vi "UMLEditor menuUpdates.vi"(0 "menu":refnum<k9>, 1 "menuAction":T1, 2 "item":string, 3 "addfirst(false)":bool, 5 "error in (no error)":errorcluster) -> (19 "error out":errorcluster)   [LabVIEW 2020]
doc: "Gets current diagram values"
uses:
  <resource>/Framework/Providers/Open_GDS/UML/UMLEditor/UMLEditor MenuActionType.ctl
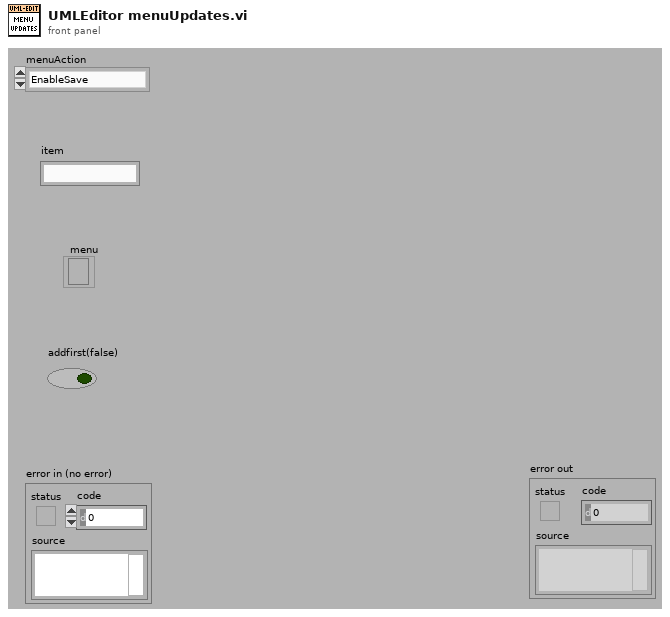
[diagram p1: front panel]
types:
  T1 = typedef "UMLEditor MenuActionType.ctl" = enum16{"EnableSave", "EnablePaste", "DisablePaste", "DiableSave", "AddRecentFile", "disablePropDel", "enablePropDel", "enablePropDisDel", "diasbleClassRel", "enableClassRel", "Class", "State", "Other", "EnableXMI", "DisableXMI", "EnableCopy", "DisableCopy"}
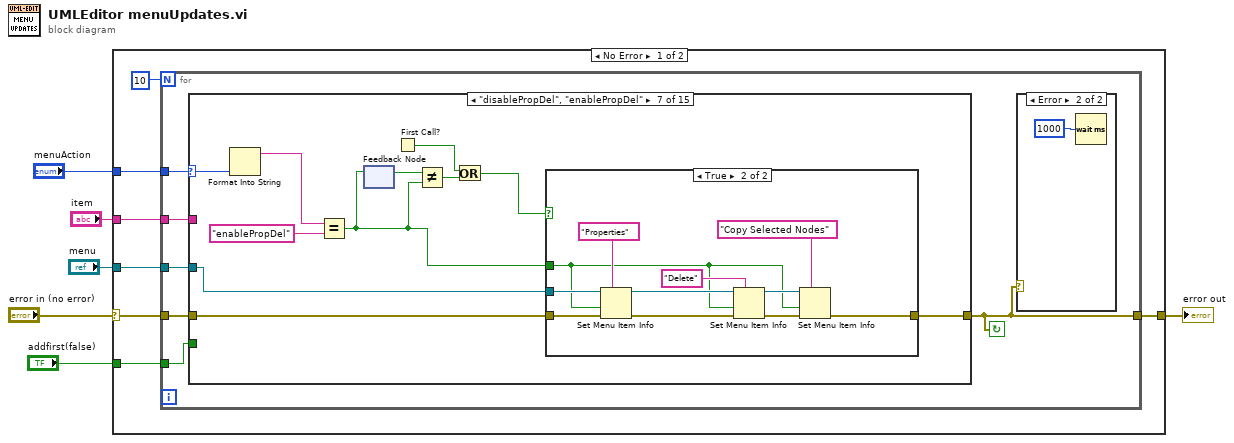
[diagram p0: block diagram]
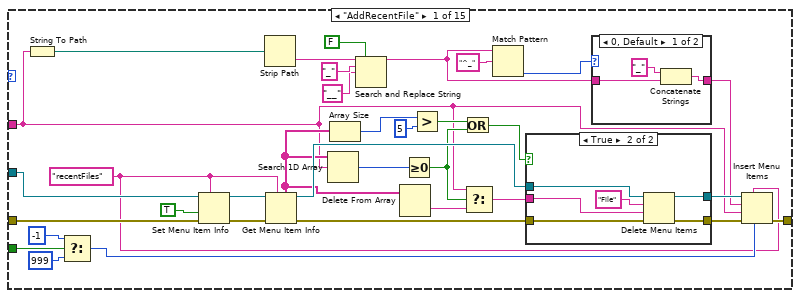
[diagram p3: hidden frame]
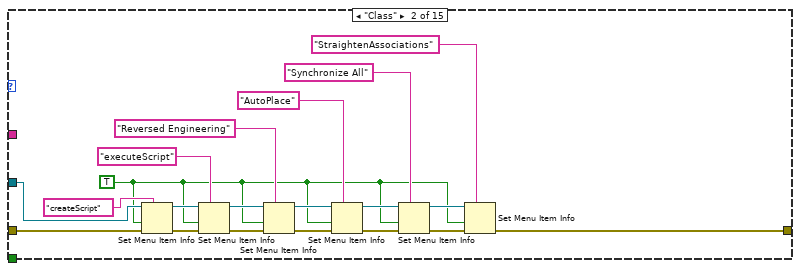
[diagram p6: hidden frame]
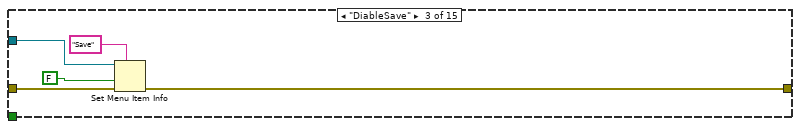
[diagram p7: hidden frame]
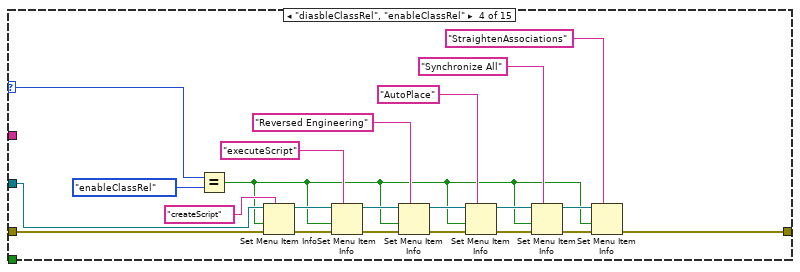
[diagram p8: hidden frame]
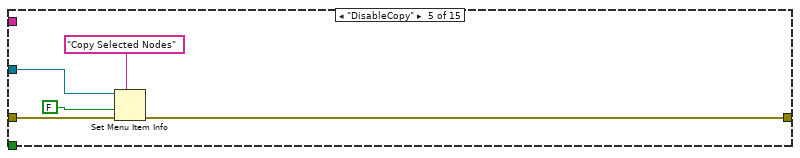
[diagram p9: hidden frame]
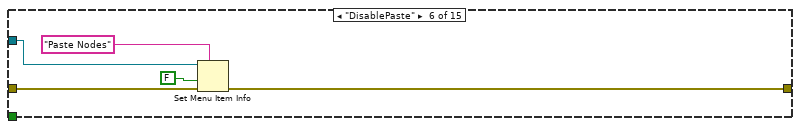
[diagram p10: hidden frame]
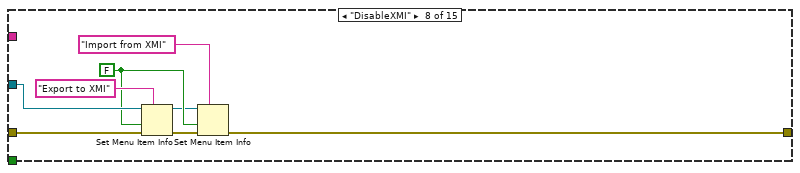
[diagram p12: hidden frame]
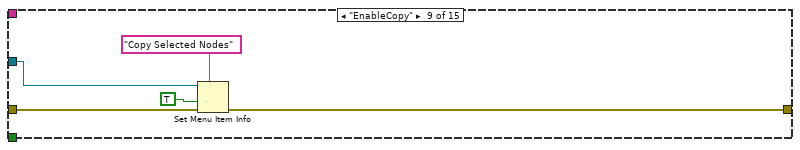
[diagram p13: hidden frame]
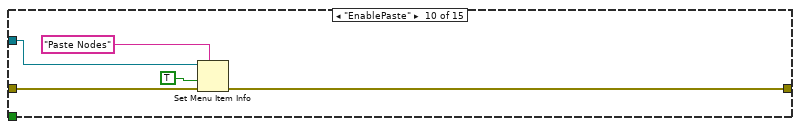
[diagram p14: hidden frame]
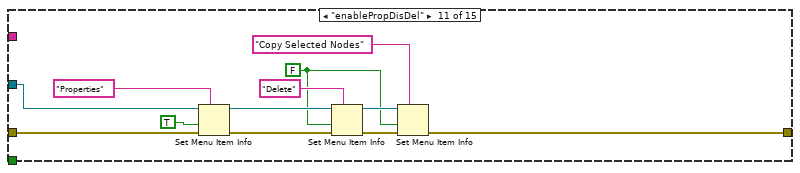
[diagram p15: hidden frame]
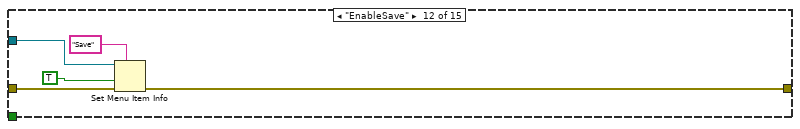
[diagram p16: hidden frame]
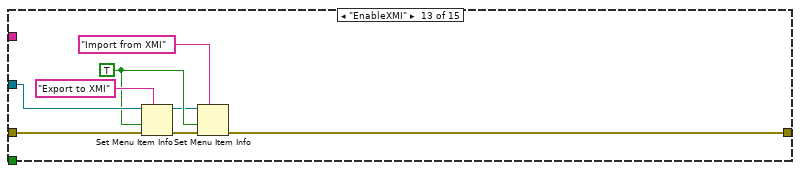
[diagram p17: hidden frame]
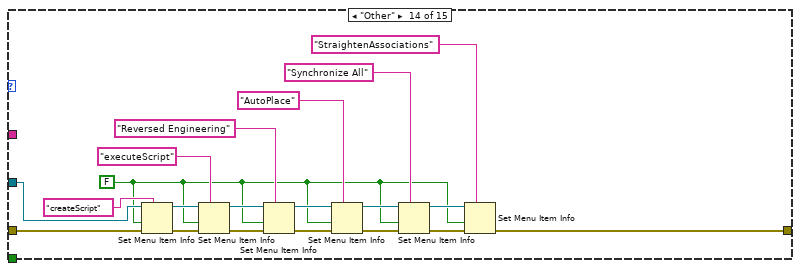
[diagram p18: hidden frame]
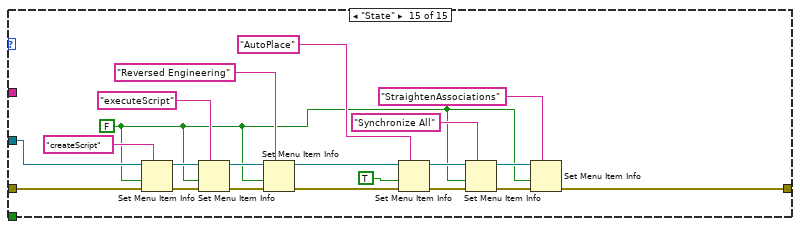
[diagram p19: hidden frame]
diagram:
  n1 = case shown="No Error" "error in (no error)" {
    selector: "error in (no error)" -> [w13 w231]
    tunnel: [w12 w231] -> w5
    tunnel: "menuAction" -> [w11 _]
    tunnel: "item" -> [w10 _]
    tunnel: "addfirst(false)" -> [w9 _]
    tunnel: "menu" -> [w8 _]
    frame No Error {
      n2 = for {
        N: 10 -> [_]
        tunnel: w11 -> [w18]
        tunnel: w10 -> [w17]
        tunnel: w9 -> [w16]
        tunnel: w8 -> [w15]
        tunnel: w13 -> [w19]
        tunnel: [w14] -> w12
        stop <- w14 continue-if-true
        n3 = case shown="\"disablePropDel\", \"enablePropDel\"" w18 {
          selector: w18 -> [_ _ _ w94 _ _ w125 _ _ _ _ _ _ _ _]
          tunnel: w15 -> [w34 w86 w91 w113 w118 w123 w134 w154 w159 w164 w176 w181 w189 w209 w230]
          tunnel: w19 -> [w32 w85 w90 w112 w117 w122 w133 w153 w158 w163 w175 w180 w188 w208 w229]
          tunnel: [w54 w68 w89 w95 w116 w121 w132 w150 w157 w162 w166 w179 w184 w191 w212] -> w14
          tunnel: w17 -> [w41 _ _ _ _ _ _ _ _ _ _ _ _ _ _]
          tunnel: w16 -> [w38 _ _ _ _ _ _ _ _ _ _ _ _ _ _]
          frame "AddRecentFile" {
            w30 = "recentFiles" ("menu tag")
            n4 = String To Path(string=w41) -> (path=w53:path)
            n5 = Select(t=-1, s=w38, f=999) -> (s? t:f=w36:i32)
            n6 = Set Menu Item Info(7:w30, 8:w32, 9:TRUE ("enabled"), 11:w34) -> (0:w31:errorcluster, 3:w33:refnum<k9>)  [unwired: 3 out]
            n7 = Strip Path(path=w53) -> (name=w28:string)  [unwired: 1 out]
            n8 = Get Menu Item Info(7:w30, 8:w31, 11:w33) -> (0:w48:errorcluster, 3:w50:refnum<k9>, 5:w46:string[])  [unwired: 4 out]
            n9 = Search 1D Array(1D array=w46, element=w41) -> (index of element=w43:i32)  [unwired: 1 out]
            n10 = Array Size(array=w46) -> (size(s)=w52:i32)
            n11 = Search and Replace String(replace all?=FALSE ("replace all? (F)"), input string=w28, search string="_", replace string="__" ("replace string (\"\")")) -> (result string=w22:string)  [unwired: 1 in, 6 out]
            n12 = Delete From Array(array=w46) -> (deleted portion=w40:string)  [unwired: 2 in, 1 out]
            n13 = Greater Or Equal To 0?(x=w43) -> (x >= 0?=w42:bool)
            n14 = Greater?(x=w52, y=5) -> (0:w44:bool)
            n15 = Or(x=w44, y=w42) -> (x .or. y?=w45:bool)
            n16 = Select(t=w41, s=w42, f=w40) -> (s? t:f=w39:string)
            n17 = Match Pattern(string=w22, regular expression="^_") -> (offset past match=w23:i32)  [unwired: 4 out]
            n18 = case shown="True" w45 {
              tunnel: w50 -> [w60 w66]
              tunnel: [w60 w65] -> w49
              tunnel: w39 -> [_ w62]
              tunnel: w48 -> [w59 w64]
              tunnel: [w59 w63] -> w47
              frame False {
              }
              frame True {
                n19 = Delete Menu Items(6:w64, 7:w62, 8:"File" ("menu tag"), 9:w66) -> (0:w63:errorcluster, 3:w65:refnum<k9>)
              }
            }
            n20 = case shown="0, Default" w23 {
              tunnel: w22 -> [w57 w58]
              tunnel: [w56 w58] -> w21
              frame 0, Default {
                n21 = Concatenate Strings("_" ("search string"), w57) -> (w56:string)
              }
              frame -1 {
              }
            }
            n22 = Insert Menu Items(4:w36, 5:w30, 6:w47, 7:w41, 8:w21, 9:w49) -> (0:w54:errorcluster)  [unwired: 2 out]
          }
          frame "Class" {
            w67 = TRUE ("enabled")
            n23 = Set Menu Item Info(7:"createScript" ("item tag"), 8:w85, 9:w67, 11:w86) -> (0:w81:errorcluster, 3:w83:refnum<k9>)  [unwired: 3 out]
            n24 = Set Menu Item Info(7:"executeScript" ("item tag"), 8:w81, 9:w67, 11:w83) -> (0:w77:errorcluster, 3:w80:refnum<k9>)  [unwired: 3 out]
            n25 = Set Menu Item Info(7:"Reversed Engineering" ("item tag"), 8:w77, 9:w67, 11:w80) -> (0:w79:errorcluster, 3:w78:refnum<k9>)  [unwired: 3 out]
            n26 = Set Menu Item Info(7:"AutoPlace" ("item tag"), 8:w79, 9:w67, 11:w78) -> (0:w73:errorcluster, 3:w72:refnum<k9>)  [unwired: 3 out]
            n27 = Set Menu Item Info(7:"Synchronize All" ("item tag"), 8:w73, 9:w67, 11:w72) -> (0:w69:errorcluster, 3:w70:refnum<k9>)  [unwired: 3 out]
            n28 = Set Menu Item Info(7:"StraightenAssociations" ("item tag"), 8:w69, 9:w67, 11:w70) -> (0:w68:errorcluster)  [unwired: 4 out]
          }
          frame "DiableSave" {
            n29 = Set Menu Item Info(7:"Save" ("item tag"), 8:w90, 9:FALSE ("enabled"), 11:w91) -> (0:w89:errorcluster)  [unwired: 4 out]
          }
          frame "diasbleClassRel", "enableClassRel" {
            n30 = Equal?(x=w94, y=UMLEditor_MenuActionType."enableClassRel") -> (x = y?=w92:bool)
            n31 = Set Menu Item Info(7:"createScript" ("item tag"), 8:w112, 9:w92, 11:w113) -> (0:w108:errorcluster, 3:w110:refnum<k9>)  [unwired: 3 out]
            n32 = Set Menu Item Info(7:"executeScript" ("item tag"), 8:w108, 9:w92, 11:w110) -> (0:w104:errorcluster, 3:w107:refnum<k9>)  [unwired: 3 out]
            n33 = Set Menu Item Info(7:"Reversed Engineering" ("item tag"), 8:w104, 9:w92, 11:w107) -> (0:w106:errorcluster, 3:w105:refnum<k9>)  [unwired: 3 out]
            n34 = Set Menu Item Info(7:"AutoPlace" ("item tag"), 8:w106, 9:w92, 11:w105) -> (0:w100:errorcluster, 3:w99:refnum<k9>)  [unwired: 3 out]
            n35 = Set Menu Item Info(7:"Synchronize All" ("item tag"), 8:w100, 9:w92, 11:w99) -> (0:w96:errorcluster, 3:w97:refnum<k9>)  [unwired: 3 out]
            n36 = Set Menu Item Info(7:"StraightenAssociations" ("item tag"), 8:w96, 9:w92, 11:w97) -> (0:w95:errorcluster)  [unwired: 4 out]
          }
          frame "DisableCopy" {
            n37 = Set Menu Item Info(7:"Copy Selected Nodes" ("item tag"), 8:w117, 9:FALSE ("enabled"), 11:w118) -> (0:w116:errorcluster)  [unwired: 4 out]
          }
          frame "DisablePaste" {
            n38 = Set Menu Item Info(7:"Paste Nodes" ("item tag"), 8:w122, 9:FALSE ("enabled"), 11:w123) -> (0:w121:errorcluster)  [unwired: 4 out]
          }
          frame "disablePropDel", "enablePropDel" {
            n39 = Format Into String(w125) -> (resulting string=w124:string)  [unwired: 3 in, 1 out]
            n40 = Equal?(x=w124, y="enablePropDel") -> (x = y?=w129:bool)
            n41 = feedback-in #1(w129) -> ()
            n42 = feedback #1() -> (w130:bool)  [unwired: 1 in]
            n43 = First Call?() -> (First Call?: T/F=w127:bool)
            n44 = Not Equal?(x=w130, y=w129) -> (x != y?=w128:bool)
            n45 = Or(x=w127, y=w128) -> (x .or. y?=w126:bool)
            n46 = case shown="True" w126 {
              tunnel: w134 -> [_ w146]
              tunnel: w133 -> [w135 w145]
              tunnel: [w135 w138] -> w132
              tunnel: w129 -> [_ w136]
              frame False {
              }
              frame True {
                n47 = Set Menu Item Info(7:"Properties" ("item tag"), 8:w145, 9:w136, 11:w146) -> (0:w141:errorcluster, 3:w143:refnum<k9>)  [unwired: 3 out]
                n48 = Set Menu Item Info(7:"Delete" ("item tag"), 8:w141, 9:w136, 11:w143) -> (0:w140:errorcluster, 3:w139:refnum<k9>)  [unwired: 3 out]
                n49 = Set Menu Item Info(7:"Copy Selected Nodes" ("item tag"), 8:w140, 9:w136, 11:w139) -> (0:w138:errorcluster)  [unwired: 4 out]
              }
            }
          }
          frame "DisableXMI" {
            w148 = FALSE ("enabled")
            n50 = Set Menu Item Info(7:"Export to XMI" ("item tag"), 8:w153, 9:w148, 11:w154) -> (0:w151:errorcluster, 3:w147:refnum<k9>)  [unwired: 3 out]
            n51 = Set Menu Item Info(7:"Import from XMI" ("item tag"), 8:w151, 9:w148, 11:w147) -> (0:w150:errorcluster)  [unwired: 4 out]
          }
          frame "EnableCopy" {
            n52 = Set Menu Item Info(7:"Copy Selected Nodes" ("item tag"), 8:w158, 9:TRUE ("enabled"), 11:w159) -> (0:w157:errorcluster)  [unwired: 4 out]
          }
          frame "EnablePaste" {
            n53 = Set Menu Item Info(7:"Paste Nodes" ("item tag"), 8:w163, 9:TRUE ("enabled"), 11:w164) -> (0:w162:errorcluster)  [unwired: 4 out]
          }
          frame "enablePropDisDel" {
            w165 = FALSE ("enabled")
            n54 = Set Menu Item Info(7:"Properties" ("item tag"), 8:w175, 9:TRUE ("enabled"), 11:w176) -> (0:w170:errorcluster, 3:w173:refnum<k9>)  [unwired: 3 out]
            n55 = Set Menu Item Info(7:"Delete" ("item tag"), 8:w170, 9:w165, 11:w173) -> (0:w168:errorcluster, 3:w167:refnum<k9>)  [unwired: 3 out]
            n56 = Set Menu Item Info(7:"Copy Selected Nodes" ("item tag"), 8:w168, 9:w165, 11:w167) -> (0:w166:errorcluster)  [unwired: 4 out]
          }
          frame "EnableSave" {
            n57 = Set Menu Item Info(7:"Save" ("item tag"), 8:w180, 9:TRUE ("enabled"), 11:w181) -> (0:w179:errorcluster)  [unwired: 4 out]
          }
          frame "EnableXMI" {
            w183 = TRUE ("enabled")
            n58 = Set Menu Item Info(7:"Export to XMI" ("item tag"), 8:w188, 9:w183, 11:w189) -> (0:w185:errorcluster, 3:w182:refnum<k9>)  [unwired: 3 out]
            n59 = Set Menu Item Info(7:"Import from XMI" ("item tag"), 8:w185, 9:w183, 11:w182) -> (0:w184:errorcluster)  [unwired: 4 out]
          }
          frame "Other" {
            w190 = FALSE ("enabled")
            n60 = Set Menu Item Info(7:"createScript" ("item tag"), 8:w208, 9:w190, 11:w209) -> (0:w204:errorcluster, 3:w206:refnum<k9>)  [unwired: 3 out]
            n61 = Set Menu Item Info(7:"executeScript" ("item tag"), 8:w204, 9:w190, 11:w206) -> (0:w200:errorcluster, 3:w203:refnum<k9>)  [unwired: 3 out]
            n62 = Set Menu Item Info(7:"Reversed Engineering" ("item tag"), 8:w200, 9:w190, 11:w203) -> (0:w202:errorcluster, 3:w201:refnum<k9>)  [unwired: 3 out]
            n63 = Set Menu Item Info(7:"AutoPlace" ("item tag"), 8:w202, 9:w190, 11:w201) -> (0:w196:errorcluster, 3:w195:refnum<k9>)  [unwired: 3 out]
            n64 = Set Menu Item Info(7:"Synchronize All" ("item tag"), 8:w196, 9:w190, 11:w195) -> (0:w192:errorcluster, 3:w193:refnum<k9>)  [unwired: 3 out]
            n65 = Set Menu Item Info(7:"StraightenAssociations" ("item tag"), 8:w192, 9:w190, 11:w193) -> (0:w191:errorcluster)  [unwired: 4 out]
          }
          frame "State" {
            w211 = FALSE ("enabled")
            n66 = Set Menu Item Info(7:"createScript" ("item tag"), 8:w229, 9:w211, 11:w230) -> (0:w225:errorcluster, 3:w227:refnum<k9>)  [unwired: 3 out]
            n67 = Set Menu Item Info(7:"executeScript" ("item tag"), 8:w225, 9:w211, 11:w227) -> (0:w221:errorcluster, 3:w224:refnum<k9>)  [unwired: 3 out]
            n68 = Set Menu Item Info(7:"Reversed Engineering" ("item tag"), 8:w221, 9:w211, 11:w224) -> (0:w223:errorcluster, 3:w222:refnum<k9>)  [unwired: 3 out]
            n69 = Set Menu Item Info(7:"AutoPlace" ("item tag"), 8:w223, 9:TRUE ("enabled"), 11:w222) -> (0:w217:errorcluster, 3:w216:refnum<k9>)  [unwired: 3 out]
            n70 = Set Menu Item Info(7:"Synchronize All" ("item tag"), 8:w217, 9:w211, 11:w216) -> (0:w213:errorcluster, 3:w214:refnum<k9>)  [unwired: 3 out]
            n71 = Set Menu Item Info(7:"StraightenAssociations" ("item tag"), 8:w213, 9:w211, 11:w214) -> (0:w212:errorcluster)  [unwired: 4 out]
          }
        }
        n72 = case shown="Error" w14 {
          frame No Error {
          }
          frame Error {
            n73 = Wait (ms)(milliseconds to wait=u32 1000) -> ()  [unwired: 1 out]
          }
        }
      }
    }
    frame Error {
    }
  }
  "error out" <- w5
